vi "Lire config LEYBOLD.vi"(2 "error in (no error)":errorcluster caption="entrée d'erreur (pas d'erreur)", 3 "refnum":T1) -> (0 "error out":errorcluster, 1 "refnum out":T1)   [LabVIEW 2022 SP3]
uses:
  <vilib>/Utility/config.llb/Config Data RefNum.ctl
  <vilib>/Utility/config.llb/Read Key (String).vi
  <vilib>/Utility/config.llb/Read Key (Boolean).vi
  Variables globales/Variable glob Leybold.vi
  <vilib>/Utility/config.llb/NI_LVConfig.lvlib
panel:
  out "Noms jauges":string[](array[string])
  out "Ports COM LEYBOLD":refnum<visa-resource-name>[](array[refnum])
  # "Lire config acqui.ini LEYBOLD"
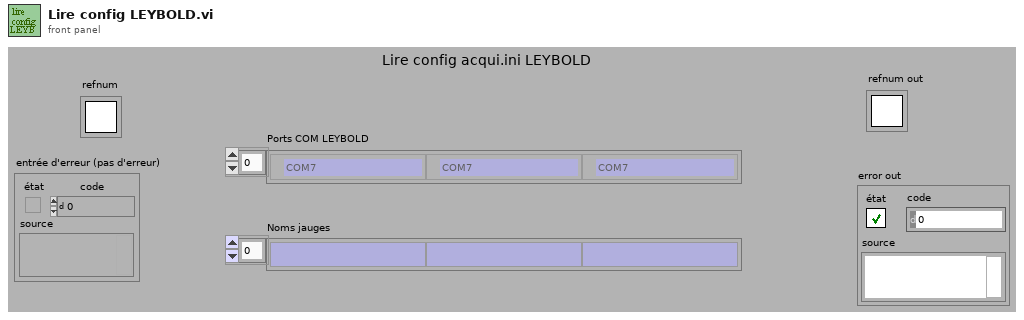
[diagram p1: front panel]
types:
  T1 = typedef "NI_LVConfig.lvlib/Config Data RefNum.ctl" = refnum<k1>
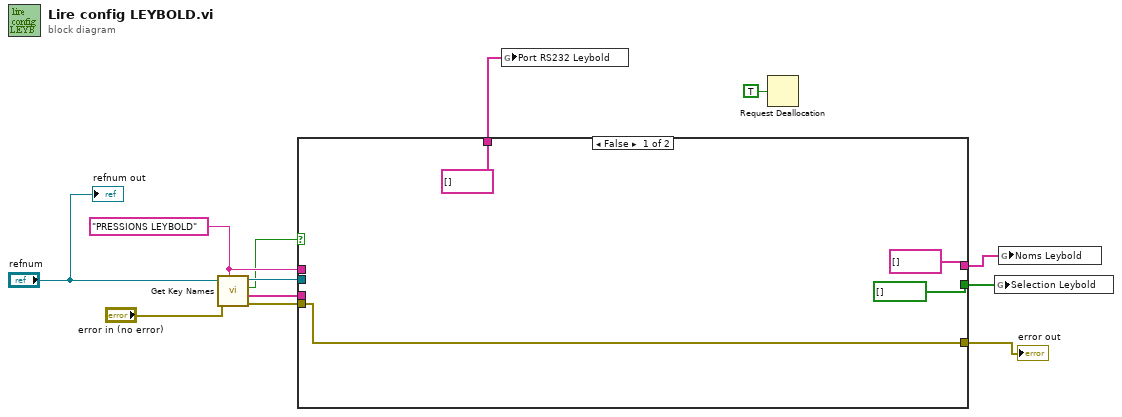
[diagram p0: block diagram]
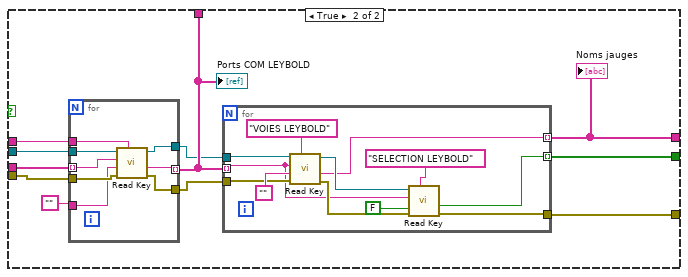
[diagram p2: hidden frame]
diagram:
  w9 = "PRESSIONS LEYBOLD" ("section")
  n1 = call <vilib>:"Get Key Names.vi"("section"=w9, "error in (no error)"="error in (no error)", "refnum"="refnum") -> ("error out"=w10:errorcluster, "key names"=w12:string[], "section exists?"=w7:bool, "refnum out"=w11:T1)  [unwired: 5 in]
  n2 = case shown="False" w7 {
    tunnel: w12 -> [_ w27]
    tunnel: w11 -> [_ w26]
    tunnel: w10 -> [w13 w25]
    tunnel: w9 -> [_ w24]
    tunnel: [bool[] [] w23] -> w3
    tunnel: [string[] [] w22] -> w5
    tunnel: [string[] [] w21] -> w4
    tunnel: [w13 w17] -> w6
    frame False {
    }
    frame True {
      n3 = for {
        tunnel: w27 -> [w44] mode=indexing
        tunnel: w26 -> [w47]
        tunnel: w25 -> [w46]
        tunnel: w24 -> [w45]
        tunnel: "" -> [w43]
        tunnel: [w42] -> w22 mode=indexing
        tunnel: [w41] -> w19
        tunnel: [w40] -> w18
        n4 = call-poly <vilib>:"Read Key.vi"("section"=w45, "error in (no error)"=w46, "default value"=w43, "key"=w44, "refnum"=w47) -> ("error out"=w40:errorcluster, "value"=w42:string, "refnum out"=w41:T1)  [unwired: 3 in, 1 out]
      }
      "Ports COM LEYBOLD" <- w22
      n5 = for {
        tunnel: w22 -> [w31] mode=indexing
        tunnel: w19 -> [w37]
        tunnel: w18 -> [w36]
        tunnel: [w33] -> w21 mode=indexing
        tunnel: [w29] -> w17
        tunnel: [w28] -> w23 mode=indexing
        n6 = call-poly <vilib>:"Read Key.vi"("section"="VOIES LEYBOLD", "error in (no error)"=w36, "default value"="", "key"=w31, "refnum"=w37) -> ("error out"=w34:errorcluster, "value"=w33:string, "refnum out"=w35:T1)  [unwired: 3 in, 1 out]
        n7 = call-poly <vilib>:"Read Key.vi"("section"="SELECTION LEYBOLD", "error in (no error)"=w34, "default value"=FALSE, "key"=w31, "refnum"=w35) -> ("error out"=w29:errorcluster, "value"=w28:bool)  [unwired: 3 in, 2 out]
      }
      "Noms jauges" <- w21
    }
  }
  "error out" <- w6
  n8 = global write "Variable glob Leybold.vi" "Port RS232 Leybold"(w5) -> ()
  n9 = Request Deallocation(TRUE ("flag")) -> ()
  n10 = global write "Variable glob Leybold.vi" "Selection Leybold"(w3) -> ()
  n11 = global write "Variable glob Leybold.vi" "Noms Leybold"(w4) -> ()
  "refnum out" <- "refnum"
